vi "Test Insertion Palette Drag Drop.vi"() -> ()   [LabVIEW 2020]
uses:
  TSnax UI/Basic UI State.ctl
  TSnax/TS License Type.ctl
  TSnax/Execution Options.ctl
  TSnax UI/SequenceViewPanel/SequenceViewPanel.lvclass
  TSnax UI/InsertionPalettePanel/InsertionPalettePanel.lvclass
  TSnax UI/TSnax UI Manager/TSnax UI Manager.lvclass
  TSnax/SequenceFile/SequenceFile.lvclass
  TSnax UI/TSnax UI.lvlib
  TSnax/TSnax.lvlib
  TSnax/Engine/Engine.lvclass
panel:
  in  "Trace Speed":u32(slide) scale=2000.0..1.0
  in  "Run SinglePass":bool
  # "Slow"
  # "Fast"
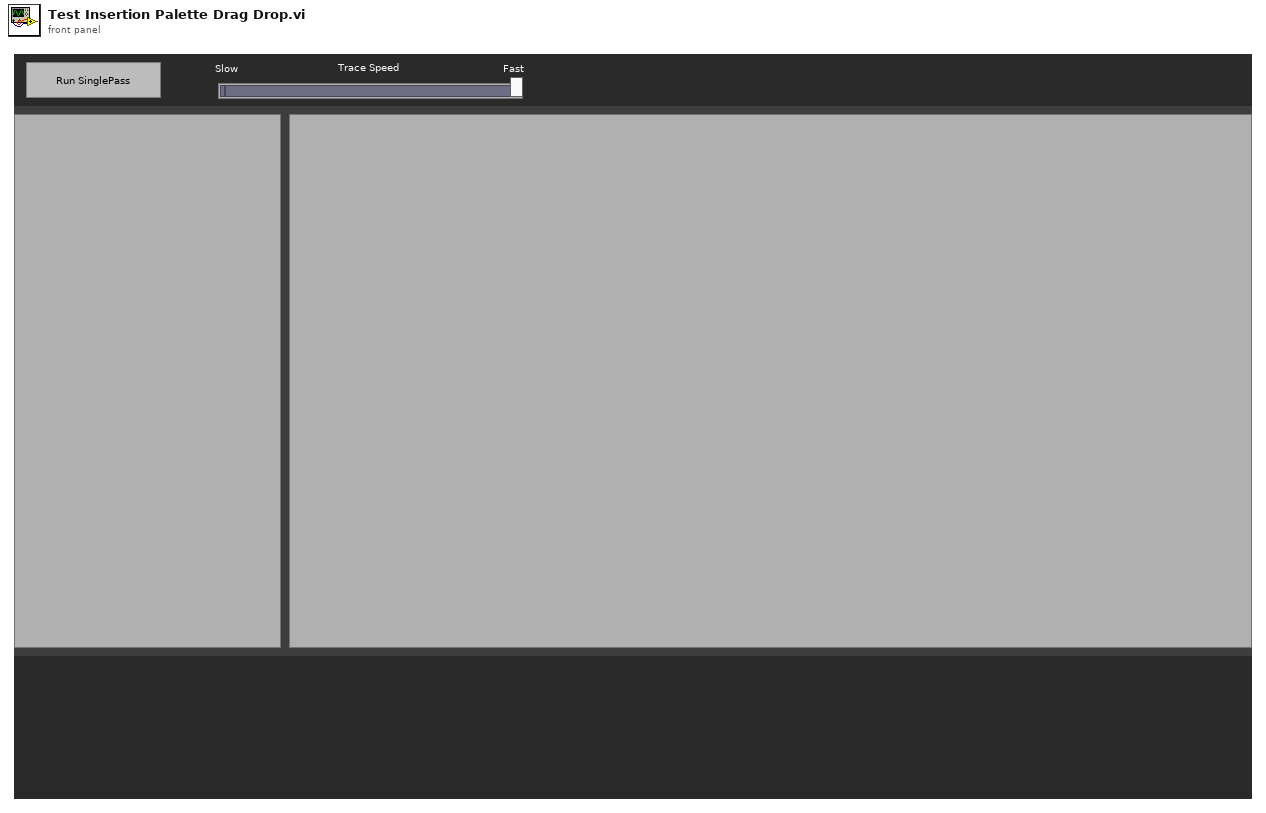
[diagram p1: front panel]
types:
  T1 = typedef "TSnax UI.lvlib/Basic UI State.ctl" = enum16{"Init", "Run", "Close"}
  T2 = typedef "TSnax.lvlib/TS License Type.ctl" = enum16{"Operator", "CustomEditor", "SequenceEditor"}
  T3 = typedef "TSnax.lvlib/Execution Options.ctl" = cluster{"Use Default Model (T)":bool, "Release Related References (T)":bool}
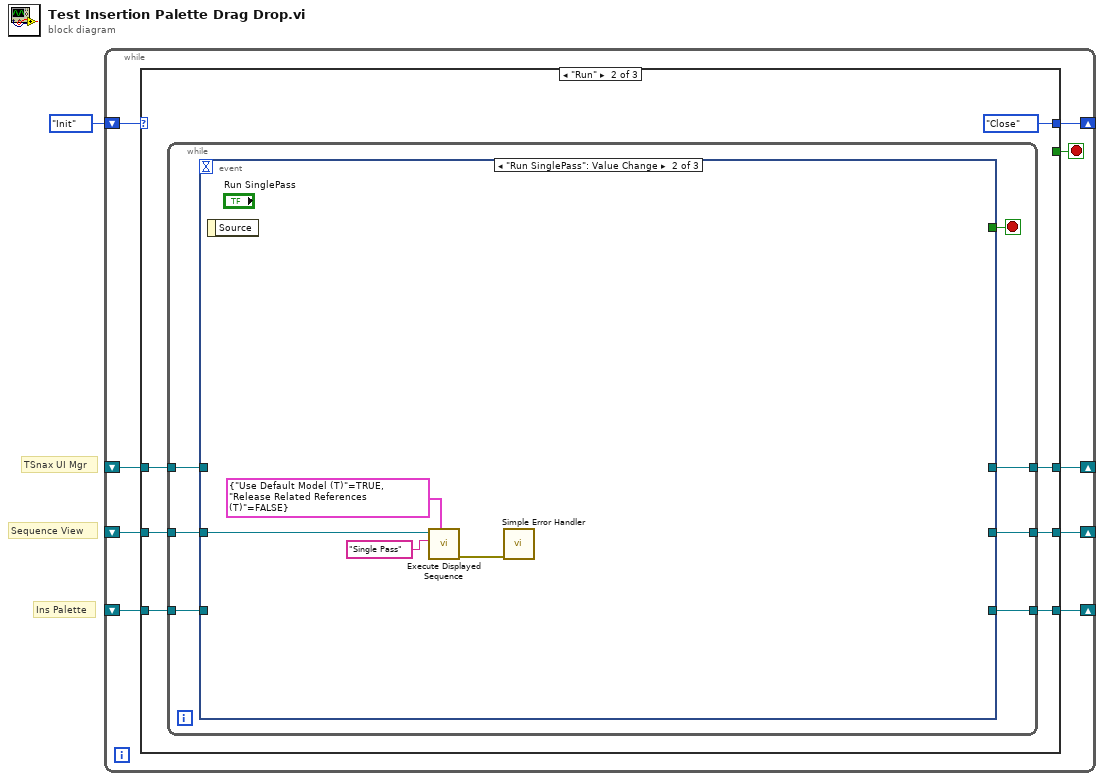
[diagram p0: block diagram]
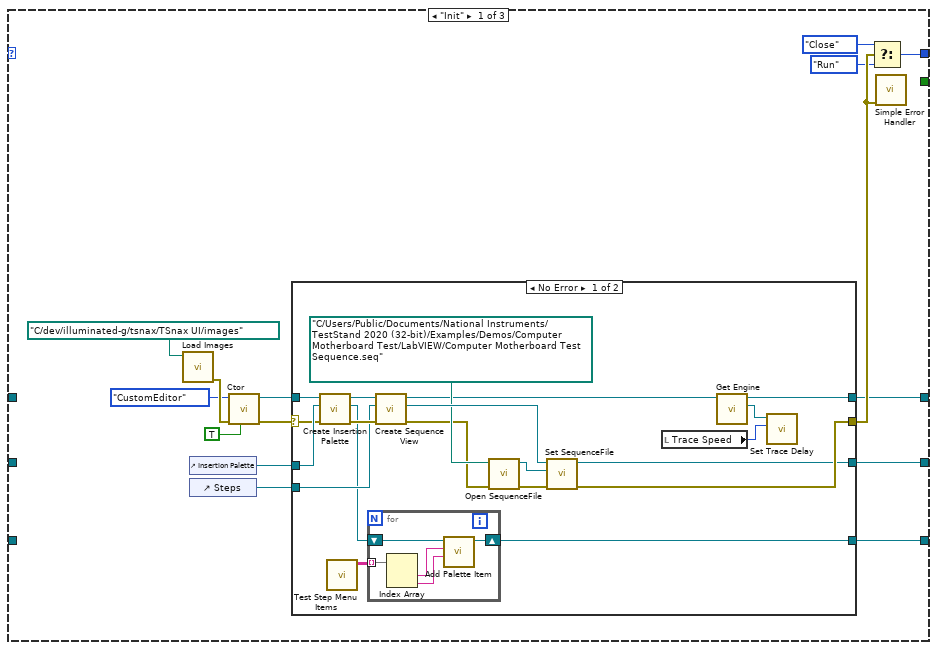
[diagram p2: hidden frame]
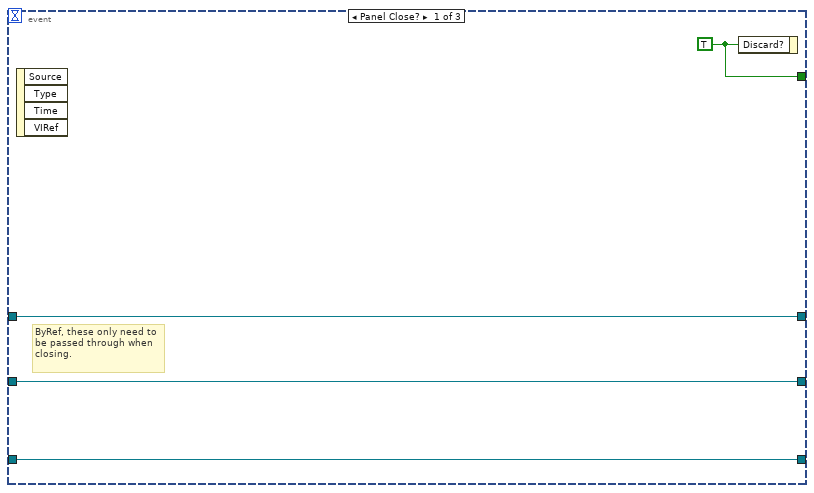
[diagram p4: hidden frame]
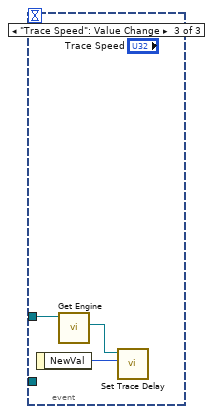
[diagram p5: hidden frame]
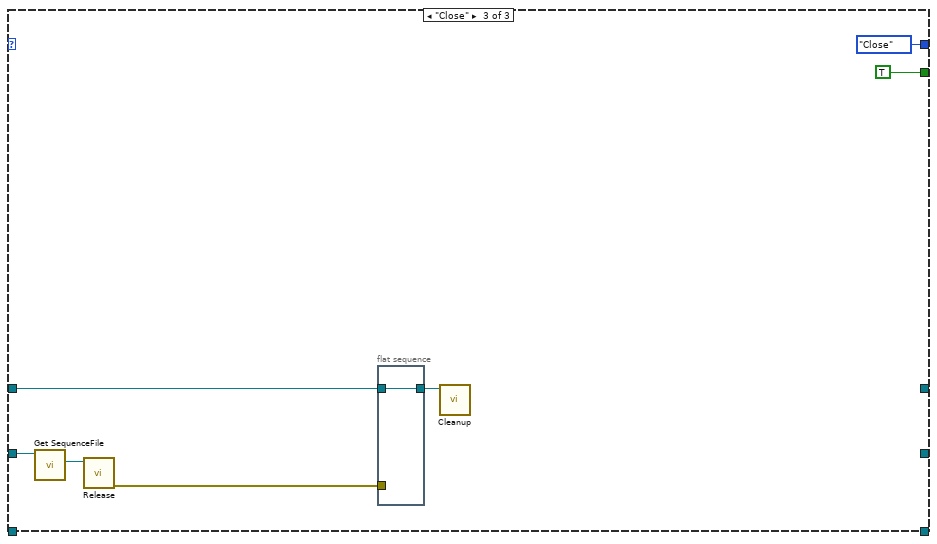
[diagram p6: hidden frame]
diagram:
  # "Ins Palette"
  # "Sequence View"
  # "TSnax UI Mgr"
  n1 = while {
    shift-right: [w9] -> _
    shift-left: Basic_UI_State."Init" ("Basic UI State") -> [w10]
    shift-right: [w7] -> _
    shift-left: _ -> [w6]
    shift-right: [w5] -> _
    shift-left: _ -> [w4]
    shift-right: [w3] -> _
    shift-left: _ -> [w2]
    stop <- w8 stop-if-true
    n2 = case shown="\"Run\"" w10 {
      tunnel: [w19 Basic_UI_State."Close" ("Basic UI State") Basic_UI_State."Close" ("Basic UI State")] -> w9
      tunnel: [_ _ TRUE] -> w8
      tunnel: [w17 w55 _] -> w7
      tunnel: w6 -> [_ w58 w79]
      tunnel: [w18 w54 _] -> w5
      tunnel: w4 -> [_ w57 w82]
      tunnel: [w23 w53 _] -> w3
      tunnel: w2 -> [_ w56 _]
      frame "Init" {
        n3 = call "Load Images.vi"("images Folder"=path "C:/dev/illuminated-g/tsnax/TSnax UI/images") -> ("error out"=w25:errorcluster)  [unwired: 10 in]
        n4 = control-ref of="Insertion Palette"() -> (w15:refnum<vi>)
        n5 = control-ref of="Steps"() -> (w16:refnum<vi>)
        n6 = call "Ctor.vi"("Debug? (F)"=TRUE, "error in (no error)"=w25, "TS License Type (Operator)"=TS_License_Type."CustomEditor") -> ("error out"=w13:errorcluster, "TSnax UI Manager out"=w14:refnum<class "TSnax UI Manager.lvclass">)  [unwired: 6 in, 1 out]
        n7 = case shown="No Error" w13 {
          selector: w13 -> [w38 w51]
          tunnel: [w45 _] -> w23
          tunnel: w14 -> [w39 w52]
          tunnel: [w34 _] -> w18
          tunnel: [w28 w52] -> w17
          tunnel: w16 -> [w41 _]
          tunnel: w15 -> [w40 _]
          tunnel: [w35 w51] -> w24
          frame No Error {
            n8 = call "Create Insertion Palette.vi"("error in (no error)"=w38, "Subpanel"=w40, "TSnax UI Manager in"=w39) -> ("error out"=w42:errorcluster, "Insertion Palette"=w37:refnum<class "InsertionPalettePanel.lvclass">, "TSnax UI Manager out"=w43:refnum<class "TSnax UI Manager.lvclass">)  [unwired: 6 in]
            n9 = call "Test Step Menu Items.vi"() -> ("Array"=w44:string[][])  [unwired: 11 in]
            n10 = for {
              shift-right: [w49] -> w45
              shift-left: w37 -> [w50]
              tunnel: w44 -> [w48] mode=indexing
              n11 = Index Array(array=w48) -> (element #1=w47:string, element #2=w46:string)  [unwired: 2 in]
              n12 = call "Add Palette Item.vi"("Group (From Step Type)"=w46, "Step Type Name"=w47, "InsertionPalettePanel in"=w50) -> ("InsertionPalettePanel out"=w49:refnum<class "InsertionPalettePanel.lvclass">)  [unwired: 7 in, 1 out]
            }
            n13 = call "Create Sequence View.vi"("error in (no error)"=w42, "Subpanel"=w41, "TSnax UI Manager in"=w43) -> ("error out"=w32:errorcluster, "Sequence View"=w36:refnum<class "SequenceViewPanel.lvclass">, "TSnax UI Manager out"=w29:refnum<class "TSnax UI Manager.lvclass">)  [unwired: 6 in]
            n14 = call "Open SequenceFile.vi"("error in (no error)"=w32, "Path"=path "C:/Users/Public/Documents/National Instruments/TestStand 2020 (32-bit)/Examples/Demos/Computer Motherboard Test/LabVIEW/Computer Motherboard Test Sequence.seq") -> ("error out"=w31:errorcluster, "SequenceFile out"=w30:refnum<class "SequenceFile.lvclass">)  [unwired: 8 in]
            n15 = call "Set SequenceFile.vi"("error in (no error)"=w31, "SequenceFile"=w30, "SequenceViewPanel in"=w36) -> ("error out"=w35:errorcluster, "SequenceViewPanel out"=w34:refnum<class "SequenceViewPanel.lvclass">)  [unwired: 7 in]
            n16 = local read "Trace Speed"() -> (w26:u32)
            n17 = call "Get Engine.vi"("TSnax UI Manager in"=w29) -> ("TSnax:Engine"=w27:refnum<class "Engine.lvclass">, "TSnax UI Manager out"=w28:refnum<class "TSnax UI Manager.lvclass">)  [unwired: 8 in, 1 out]
            n18 = call "Set Trace Delay.vi"("Trace Delay ms"=w26, "Engine in"=w27) -> ()  [unwired: 8 in, 2 out]
          }
          frame Error {
          }
        }
        n19 = Select(t=Basic_UI_State."Close" ("Basic UI State"), s=w24, f=Basic_UI_State."Run") -> (s? t:f=w19:T1)
        n20 = call <vilib>:"Simple Error Handler.vi"("error in (no error)"=w24) -> ()  [unwired: 4 in, 5 out]
      }
      frame "Run" {
        n21 = while {
          tunnel: w58 -> [w66]
          tunnel: w57 -> [w65]
          tunnel: w56 -> [w64]
          tunnel: [w62] -> w55
          tunnel: [w61] -> w54
          tunnel: [w60] -> w53
          stop <- w63 stop-if-true
          n22 = event shown="[1] \"Run SinglePass\": Value Change" {
            selector: _ -> [_ _ _]
            dyn-events: _ -> [_ _ _]
            timeout: _ -> [_ _ _]
            tunnel: w66 -> [w69 _ w76]
            tunnel: w65 -> [w68 w74 _]
            tunnel: w64 -> [w67 _ _]
            tunnel: [w70 _ _] -> w63
            tunnel: [w69 _ _] -> w62
            tunnel: [w68 _ _] -> w61
            tunnel: [w67 _ _] -> w60
            event Panel Close? {
              w70 = TRUE ("Discard?")
              # "ByRef, these only need to be passed through when closing."
              n23 = event-data() -> ()  [unwired: 1 in, 4 out]
              n24 = event-data("Discard?"=w70) -> ()  [unwired: 1 in, 1 out]
            }
            event "Run SinglePass": Value Change {
              n25 = event-data() -> ()  [unwired: 1 in, 1 out]
              n26 = call "Execute Displayed Sequence.vi"("Execution Options (Default)"=T3 {"Use Default Model (T)"=TRUE, "Release Related References (T)"=FALSE}, "Entry Point"="Single Pass" ("Entry Sequence"), "SequenceViewPanel in"=w74) -> ("error out"=w71:errorcluster)  [unwired: 6 in, 2 out]
              n27 = call <vilib>:"Simple Error Handler.vi"("error in (no error)"=w71) -> ()  [unwired: 4 in, 5 out]
            }
            event "Trace Speed": Value Change {
              n28 = event-data() -> ("NewVal"=w77:u32)  [unwired: 1 in]
              n29 = call "Get Engine.vi"("TSnax UI Manager in"=w76) -> ("TSnax:Engine"=w75:refnum<class "Engine.lvclass">)  [unwired: 8 in, 2 out]
              n30 = call "Set Trace Delay.vi"("Trace Delay ms"=w77, "Engine in"=w75) -> ()  [unwired: 8 in, 2 out]
            }
          }
        }
      }
      frame "Close" {
        n31 = call "Get SequenceFile.vi"("SequenceViewPanel in"=w82) -> ("SequenceFile"=w81:refnum<class "SequenceFile.lvclass">)  [unwired: 8 in, 2 out]
        n32 = call-dynamic "Release.vi"("SequenceFile in"=w81) -> ("error out"=w80:errorcluster)  [unwired: 10 in]
        n33 = flat-sequence {
          tunnel: w80 -> [_]
          tunnel: w79 -> [w85]
          tunnel: [w85] -> w78
          frame #0 {
          }
        }
        n34 = call "Cleanup.vi"("TSnax UI Manager in"=w78) -> ()  [unwired: 10 in, 1 out]
      }
    }
  }
